vi "Module Init.vi"(8 "error in (no error)":errorcluster, 11 "Data Processor Module in":refnum<class "Data Processor Module.lvclass">) -> (0 "error out":errorcluster, 3 "Data Processor Module out":refnum<class "Data Processor Module.lvclass">)   [LabVIEW 2020, in "VolatusData.lvlib" / "Data Processor Module.lvclass"]
uses:
  Data Processor Module.lvclass
  C:/dev/lv20CE/relink/lv-volatus/Volatus/Module/Module.lvclass
  Volatus/Module/Module.lvclass/Module.ctl
  Volatus/MessageQ/MessageQ.lvclass/MessageQ.ctl
  Volatus/Module/Self Q.vi
  Volatus/MessageQ/Send.vi
  Volatus/Module/Module.lvclass
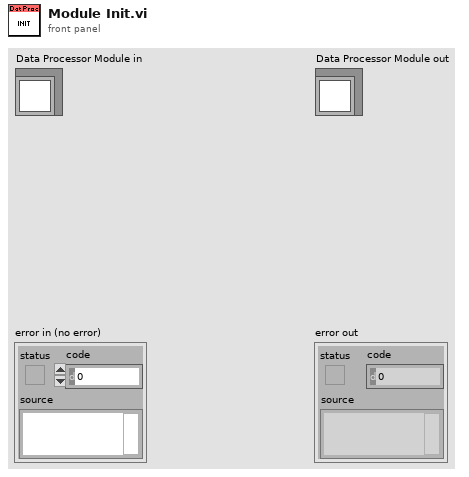
[diagram p1: front panel]
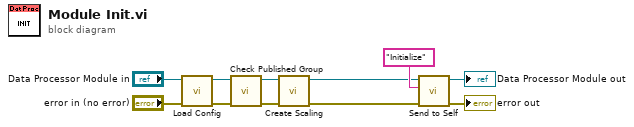
[diagram p0: block diagram]
diagram:
  n1 = call "Load Config.vi"("error in (no error)"="error in (no error)", "Data Processor Module in"="Data Processor Module in") -> ("error out"=w3:errorcluster, "Data Processor Module out"=w1:refnum<class "Data Processor Module.lvclass">)  [unwired: 8 in]
  n2 = call "Check Published Group.vi"("error in (no error)"=w3, "Data Processor Module in"=w1) -> ("error out"=w10:errorcluster, "Data Processor Module out"=w9:refnum<class "Data Processor Module.lvclass">)  [unwired: 8 in]
  n3 = call "Create Scaling.vi"("error in (no error)"=w10, "Data Processor Module in"=w9) -> ("error out"=w6:errorcluster, "Data Processor Module out"=w7:refnum<class "Data Processor Module.lvclass">)  [unwired: 8 in]
  n4 = call "Send to Self.vi"("error in (no error)"=w6, "Message ID"="Initialize", "Module in"=w7) -> ("error out"=→"error out":errorcluster, "Module out"=→"Data Processor Module out":refnum<class "Data Processor Module.lvclass">)  [unwired: 7 in]
